vi "Init Module.vi"(7 "Create from class input? (F)":bool, 8 "error in (no error)":errorcluster, 9 "RSI Module in":refnum<class "RSI Module.lvclass">, 10 "Slot Settings":T1, 11 "Module Model":T2) -> (0 "error out":errorcluster, 3 "RSI Module out":refnum<class "RSI Module.lvclass">)   [LabVIEW 2020, in "Modules.lvlib"]
uses:
  Modules.lvlib
  RSI Module/Module Models.ctl
  RSI Module/Slot Settings.ctl
  RSI Module/RSI Module.lvclass
  RSI Module/Channels.ctl
  RSI Module/Channel Type.ctl
  9213/9213.lvclass
  C:/Users/nitest/Desktop/Git 2020/niveristand-scan-engine-module-libraries/Source/RSI Module/RSI Module.lvclass
  9203/9203.lvclass
  9205/9205.lvclass
  9207/9207.lvclass
  9209/9209.lvclass
  9210/9210.lvclass
  9211/9211.lvclass
  9212/9212.lvclass
  9214/9214.lvclass
  9216/9216.lvclass
  9217/9217.lvclass
  9219/9219.lvclass
  9224/9224.lvclass
  9226/9226.lvclass
  9229/9229.lvclass
  9233/9233.lvclass
  9234/9234.lvclass
  9235/9235.lvclass
  9237/9237.lvclass
  9239/9239.lvclass
  9242/9242.lvclass
  9244/9244.lvclass
  9253/9253.lvclass
  9350/9350.lvclass
  9401/9401.lvclass
  9402/9402.lvclass
  9403/9403.lvclass
  9478/9478.lvclass
  SD Module/SD Module.lvclass
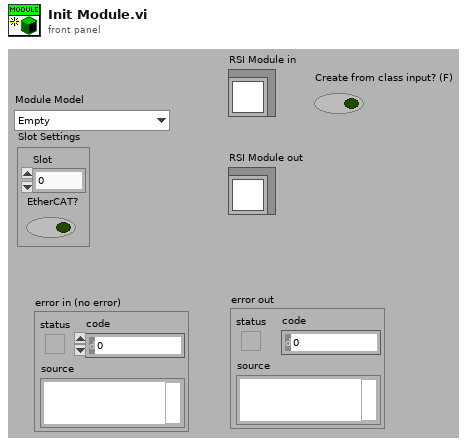
[diagram p1: front panel]
types:
  T1 = typedef "Modules.lvlib/RSI Module.lvclass/Slot Settings.ctl" = cluster{"Slot":u32, "EtherCAT?":bool}
  T2 = typedef "Modules.lvlib/RSI Module.lvclass/Module Models.ctl" = enum16{"Empty", "NI 9201", "NI 9203", "NI 9205", "NI 9206", "NI 9207", "NI 9208", "NI 9209", "NI 9210", "NI 9211", "NI 9212", "NI 9213", "NI 9214", "NI 9215", "NI 9216", "NI 9217", "NI 9219", "NI 9220", "NI 9221", "NI 9222", "NI 9223", "NI 9224", "NI 9225", "NI 9226", "NI 9227", "NI 9228", "NI 9229", "NI 9233", "NI 9234", "NI 9235", "NI 9236", "NI 9237", "NI 9239", "NI 9242", "NI 9244", "NI 9253", "NI 9263", "NI 9264", "NI 9265", "NI 9266", "NI 9269", "NI 9344", "NI 9350", "NI 9375", "NI 9401", "NI 9402", "NI 9403", "NI 9411", "NI 9421", "NI 9422", "NI 9423", "NI 9425", "NI 9426", "NI 9435", "NI 9436", "NI 9437", "NI 9472", "NI 9474", "NI 9475", "NI 9476", "NI 9477", "NI 9478", "NI 9481", "NI 9482", "NI 9485"}
  T3 = typedef "Modules.lvlib/RSI Module.lvclass/Channels.ctl" = cluster{"# Input Channels":i32, "# Output Channels":i32, "Channel Type":T4, "Units":string}
  T4 = typedef "Modules.lvlib/RSI Module.lvclass/Channel Type.ctl" = enum16{"Analog", "Digital"}
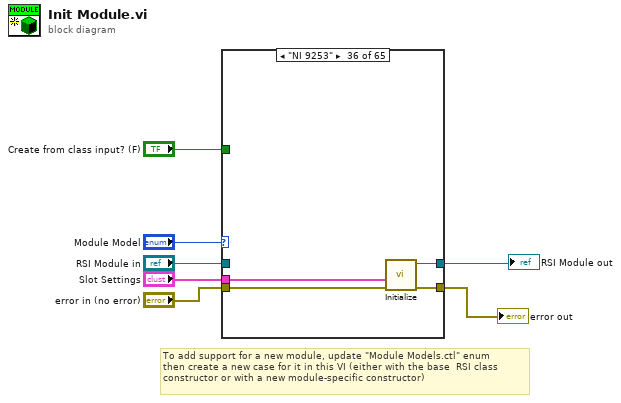
[diagram p0: block diagram]
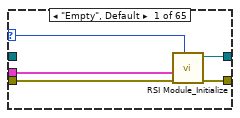
[diagram p2: hidden frame]
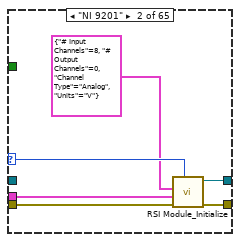
[diagram p3: hidden frame]
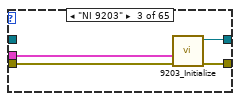
[diagram p4: hidden frame]
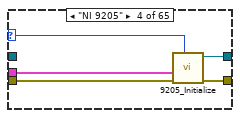
[diagram p5: hidden frame]
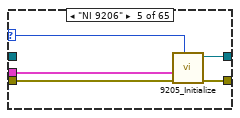
[diagram p6: hidden frame]
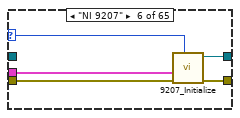
[diagram p7: hidden frame]
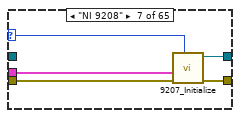
[diagram p8: hidden frame]
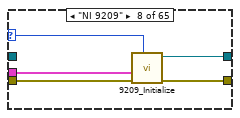
[diagram p9: hidden frame]
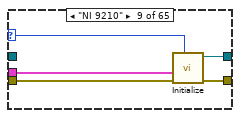
[diagram p10: hidden frame]
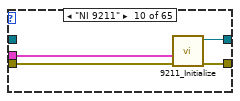
[diagram p11: hidden frame]
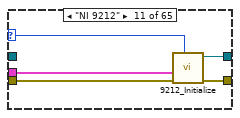
[diagram p12: hidden frame]
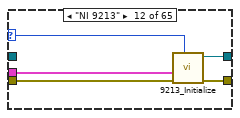
[diagram p13: hidden frame]
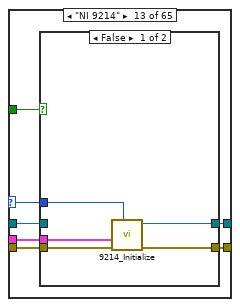
[diagram p14: hidden frame]
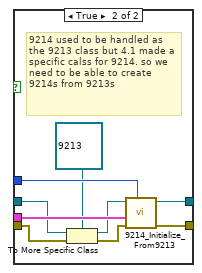
[diagram p15: hidden frame]
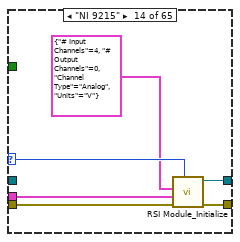
[diagram p16: hidden frame]
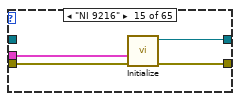
[diagram p17: hidden frame]
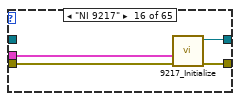
[diagram p18: hidden frame]
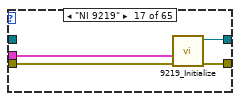
[diagram p19: hidden frame]
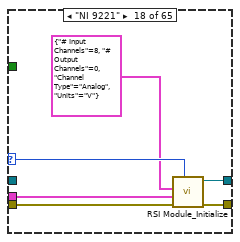
[diagram p20: hidden frame]
diagram:
  # "To add support for a new module, update \"Module Models.ctl\" enum\nthen create a new case for it in this VI (either with the base  RSI class\nconstructor or with a new module-specific constructor)"
  n1 = case shown="\"NI 9253\"" "Module Model" {
    selector: "Module Model" -> [w8 w18 _ w23 w29 w33 w38 w43 w48 _ w57 w62 w69 w93 _ _ _ w111 w117 w123 w129 w134 w140 _ w150 w155 _ _ _ w168 w173 _ _ _ _ _ w203 w209 w215 w221 w227 w233 w235 w244 _ _ _ w263 w279 w297 w317 w338 w344 w347 w366 w386 w404 w421 w442 w464 w470 _ w480 w486 w492]
    tunnel: [w11 w17 w19 w25 w31 w35 w40 w47 w51 w54 w60 w65 w72 w92 w97 w101 w105 w110 w116 w122 w128 w133 w139 w144 w149 w154 w158 w162 w167 w172 w177 w179 w184 w186 w190 w194 w202 w208 w214 w220 w226 w232 w236 w243 w248 w252 w256 w262 w281 w299 w319 w337 w343 w350 w369 w388 w407 w426 w445 w463 w469 w473 w479 w485 w491] -> w3
    tunnel: [w12 w16 w22 w26 w32 w36 w41 w46 w52 w55 w61 w66 w73 w91 w96 w100 w104 w109 w115 w121 w127 w132 w138 w143 w148 w153 w159 w163 w166 w169 w174 w178 w185 w189 w193 w197 w201 w207 w213 w219 w225 w231 w237 w242 w247 w251 w255 w261 w280 w300 w314 w336 w342 w349 w368 w387 w406 w425 w444 w462 w468 w474 w478 w484 w490] -> w6
    tunnel: "Slot Settings" -> [w9 w14 w20 w27 w28 w37 w42 w44 w49 w56 w58 w63 w70 w89 w95 w99 w103 w107 w113 w119 w125 w131 w136 w142 w146 w152 w156 w161 w165 w170 w175 w180 w182 w187 w191 w195 w199 w205 w211 w217 w223 w229 w234 w240 w246 w250 w254 w258 w277 w296 w316 w334 w340 w346 w365 w384 w402 w423 w440 w460 w466 w471 w476 w482 w488]
    tunnel: "error in (no error)" -> [w10 w13 w21 w24 w30 w34 w39 w45 w50 w53 w59 w64 w71 w88 w94 w98 w102 w106 w112 w118 w124 w130 w135 w141 w145 w151 w157 w160 w164 w171 w176 w181 w183 w188 w192 w196 w198 w204 w210 w216 w222 w228 w238 w239 w245 w249 w253 w259 w278 w295 w315 w333 w339 w345 w364 w385 w403 w424 w441 w459 w465 w472 w475 w481 w487]
    tunnel: "Create from class input? (F)" -> [_ _ _ _ _ _ _ _ _ _ _ _ w68 _ _ _ _ _ _ _ _ _ _ _ _ _ _ _ _ _ _ _ _ _ _ _ _ _ _ _ _ _ _ _ _ _ _ _ _ _ _ _ _ _ _ _ _ _ _ _ _ _ _ _ _]
    tunnel: "RSI Module in" -> [_ _ _ _ _ _ _ _ _ _ _ _ w67 _ _ _ _ _ _ _ _ _ _ _ _ _ _ _ _ _ _ _ _ _ _ _ _ _ _ _ _ _ _ _ _ _ _ _ _ _ _ _ _ _ _ _ _ _ _ _ _ _ _ _ _]
    frame "Empty", Default {
      n2 = call "RSI Module_Initialize.vi"("Module Model"=w8, "error in (no error)"=w10, "Slot Settings"=w9) -> ("error out"=w12:errorcluster, "RSI Module out"=w11:refnum<class "RSI Module.lvclass">)  [unwired: 7 in]
    }
    frame "NI 9201" {
      n3 = call "RSI Module_Initialize.vi"("Module Model"=w18, "error in (no error)"=w13, "Slot Settings"=w14, "Channels"=T3 {"# Input Channels"=8, "# Output Channels"=0, "Channel Type"=enum."Analog", "Units"="V"}) -> ("error out"=w16:errorcluster, "RSI Module out"=w17:refnum<class "RSI Module.lvclass">)  [unwired: 6 in]
    }
    frame "NI 9203" {
      n4 = call "9203_Initialize.vi"("error in (no error)"=w21, "Slot Settings"=w20) -> ("error out"=w22:errorcluster, "9203 out"=w19:refnum<class "9203.lvclass">)  [unwired: 8 in]
    }
    frame "NI 9205" {
      n5 = call "9205_Initialize.vi"("Module Model"=w23, "error in (no error)"=w24, "Slot Settings"=w27) -> ("error out"=w26:errorcluster, "9205 out"=w25:refnum<class "9205.lvclass">)  [unwired: 7 in]
    }
    frame "NI 9206" {
      n6 = call "9205_Initialize.vi"("Module Model"=w29, "error in (no error)"=w30, "Slot Settings"=w28) -> ("error out"=w32:errorcluster, "9205 out"=w31:refnum<class "9205.lvclass">)  [unwired: 7 in]
    }
    frame "NI 9207" {
      n7 = call "9207_Initialize.vi"("Module Model"=w33, "error in (no error)"=w34, "Slot Settings"=w37) -> ("error out"=w36:errorcluster, "9207 out"=w35:refnum<class "9207.lvclass">)  [unwired: 7 in]
    }
    frame "NI 9208" {
      n8 = call "9207_Initialize.vi"("Module Model"=w38, "error in (no error)"=w39, "Slot Settings"=w42) -> ("error out"=w41:errorcluster, "9207 out"=w40:refnum<class "9207.lvclass">)  [unwired: 7 in]
    }
    frame "NI 9209" {
      n9 = call "9209_Initialize.vi"("Module Model"=w43, "error in (no error)"=w45, "Slot Settings"=w44) -> ("error out"=w46:errorcluster, "9209 out"=w47:refnum<class "9209.lvclass">)  [unwired: 7 in]
    }
    frame "NI 9210" {
      n10 = call "Initialize.vi"("Module Model"=w48, "error in"=w50, "Slot Settings"=w49) -> ("error out"=w52:errorcluster, "9210 out"=w51:refnum<class "9210.lvclass">)  [unwired: 7 in]
    }
    frame "NI 9211" {
      n11 = call "9211_Initialize.vi"("error in (no error)"=w53, "Slot Settings"=w56) -> ("error out"=w55:errorcluster, "9211 out"=w54:refnum<class "9211.lvclass">)  [unwired: 8 in]
    }
    frame "NI 9212" {
      n12 = call "9212_Initialize.vi"("Module Model"=w57, "error in (no error)"=w59, "Slot Settings"=w58) -> ("error out"=w61:errorcluster, "9213 out"=w60:refnum<class "9212.lvclass">)  [unwired: 7 in]
    }
    frame "NI 9213" {
      n13 = call "9213_Initialize.vi"("Module Model"=w62, "error in (no error)"=w64, "Slot Settings"=w63) -> ("error out"=w66:errorcluster, "9213 out"=w65:refnum<class "9213.lvclass">)  [unwired: 7 in]
    }
    frame "NI 9214" {
      n14 = case shown="False" w68 {
        tunnel: [w78 w87] -> w73
        tunnel: [w77 w86] -> w72
        tunnel: w71 -> [w76 w83]
        tunnel: w70 -> [w75 w85]
        tunnel: w69 -> [w74 w84]
        tunnel: w67 -> [_ w82]
        frame False {
          n15 = call "9214_Initialize.vi"("Module Model"=w74, "error in (no error)"=w76, "Slot Settings"=w75) -> ("error out"=w78:errorcluster, "9214 out"=w77:refnum<class "9214.lvclass">)  [unwired: 7 in]
        }
        frame True {
          # "9214 used to be handled as the 9213 class but 4.1 made a specific calss for 9214. so we need to be able to create 9214s from 9213s"
          n16 = To More Specific Class(target class=refnum<class "9213.lvclass"> refnum ("Modules.lvlib:9213.lvclass"), reference=w82, error in=w83) -> (specific class reference=w80:refnum<class "9213.lvclass">, error out=w79:errorcluster)
          n17 = call "9214_Initialize_From9213.vi"("Module Model"=w84, "error in (no error)"=w79, "Slot Settings"=w85, "9213 in"=w80) -> ("error out"=w87:errorcluster, "9214 out"=w86:refnum<class "9214.lvclass">)  [unwired: 6 in]
        }
      }
    }
    frame "NI 9215" {
      n18 = call "RSI Module_Initialize.vi"("Module Model"=w93, "error in (no error)"=w88, "Slot Settings"=w89, "Channels"=T3 {"# Input Channels"=4, "# Output Channels"=0, "Channel Type"=enum."Analog", "Units"="V"}) -> ("error out"=w91:errorcluster, "RSI Module out"=w92:refnum<class "RSI Module.lvclass">)  [unwired: 6 in]
    }
    frame "NI 9216" {
      n19 = call "Initialize.vi"("error in"=w94, "Slot Settings"=w95) -> ("error out"=w96:errorcluster, "9216 out"=w97:refnum<class "9216.lvclass">)  [unwired: 8 in]
    }
    frame "NI 9217" {
      n20 = call "9217_Initialize.vi"("error in (no error)"=w98, "Slot Settings"=w99) -> ("error out"=w100:errorcluster, "9217 out"=w101:refnum<class "9217.lvclass">)  [unwired: 8 in]
    }
    frame "NI 9219" {
      n21 = call "9219_Initialize.vi"("error in (no error)"=w102, "Slot Settings"=w103) -> ("error out"=w104:errorcluster, "9219 out"=w105:refnum<class "9219.lvclass">)  [unwired: 8 in]
    }
    frame "NI 9221" {
      n22 = call "RSI Module_Initialize.vi"("Module Model"=w111, "error in (no error)"=w106, "Slot Settings"=w107, "Channels"=T3 {"# Input Channels"=8, "# Output Channels"=0, "Channel Type"=enum."Analog", "Units"="V"}) -> ("error out"=w109:errorcluster, "RSI Module out"=w110:refnum<class "RSI Module.lvclass">)  [unwired: 6 in]
    }
    frame "NI 9220" {
      n23 = call "RSI Module_Initialize.vi"("Module Model"=w117, "error in (no error)"=w112, "Slot Settings"=w113, "Channels"=T3 {"# Input Channels"=16, "# Output Channels"=0, "Channel Type"=enum."Analog", "Units"="V"}) -> ("error out"=w115:errorcluster, "RSI Module out"=w116:refnum<class "RSI Module.lvclass">)  [unwired: 6 in]
    }
    frame "NI 9222" {
      n24 = call "RSI Module_Initialize.vi"("Module Model"=w123, "error in (no error)"=w118, "Slot Settings"=w119, "Channels"=T3 {"# Input Channels"=4, "# Output Channels"=0, "Channel Type"=enum."Analog", "Units"="V"}) -> ("error out"=w121:errorcluster, "RSI Module out"=w122:refnum<class "RSI Module.lvclass">)  [unwired: 6 in]
    }
    frame "NI 9223" {
      n25 = call "RSI Module_Initialize.vi"("Module Model"=w129, "error in (no error)"=w124, "Slot Settings"=w125, "Channels"=T3 {"# Input Channels"=4, "# Output Channels"=0, "Channel Type"=enum."Analog", "Units"="V"}) -> ("error out"=w127:errorcluster, "RSI Module out"=w128:refnum<class "RSI Module.lvclass">)  [unwired: 6 in]
    }
    frame "NI 9224" {
      n26 = call "9224_Initialize.vi"("Module Model"=w134, "error in (no error)"=w130, "Slot Settings"=w131) -> ("error out"=w132:errorcluster, "9224 out"=w133:refnum<class "9224.lvclass">)  [unwired: 7 in]
    }
    frame "NI 9225" {
      n27 = call "RSI Module_Initialize.vi"("Module Model"=w140, "error in (no error)"=w135, "Slot Settings"=w136, "Channels"=T3 {"# Input Channels"=3, "# Output Channels"=0, "Channel Type"=enum."Analog", "Units"="Vrms"}) -> ("error out"=w138:errorcluster, "RSI Module out"=w139:refnum<class "RSI Module.lvclass">)  [unwired: 6 in]
    }
    frame "NI 9226" {
      n28 = call "Initialize.vi"("error in"=w141, "Slot Settings"=w142) -> ("error out"=w143:errorcluster, "9226 out"=w144:refnum<class "9226.lvclass">)  [unwired: 8 in]
    }
    frame "NI 9227" {
      n29 = call "RSI Module_Initialize.vi"("Module Model"=w150, "error in (no error)"=w145, "Slot Settings"=w146, "Channels"=T3 {"# Input Channels"=4, "# Output Channels"=0, "Channel Type"=enum."Analog", "Units"="Arms"}) -> ("error out"=w148:errorcluster, "RSI Module out"=w149:refnum<class "RSI Module.lvclass">)  [unwired: 6 in]
    }
    frame "NI 9228" {
      n30 = call "9224_Initialize.vi"("Module Model"=w155, "error in (no error)"=w151, "Slot Settings"=w152) -> ("error out"=w153:errorcluster, "9224 out"=w154:refnum<class "9224.lvclass">)  [unwired: 7 in]
    }
    frame "NI 9229" {
      n31 = call "9229_Initialize.vi"("error in (no error)"=w157, "Slot Settings"=w156) -> ("error out"=w159:errorcluster, "9229 out"=w158:refnum<class "9229.lvclass">)  [unwired: 8 in]
    }
    frame "NI 9233" {
      n32 = call "9233_Initialize.vi"("error in (no error)"=w160, "Slot Settings"=w161) -> ("error out"=w163:errorcluster, "9233 out"=w162:refnum<class "9233.lvclass">)  [unwired: 8 in]
    }
    frame "NI 9234" {
      n33 = call "9234_Initialize.vi"("error in (no error)"=w164, "Slot Settings"=w165) -> ("error out"=w166:errorcluster, "9234 out"=w167:refnum<class "9234.lvclass">)  [unwired: 8 in]
    }
    frame "NI 9235" {
      n34 = call "9235_Initialize.vi"("Module Model"=w168, "error in (no error)"=w171, "Slot Settings"=w170) -> ("error out"=w169:errorcluster, "9235 out"=w172:refnum<class "9235.lvclass">)  [unwired: 7 in]
    }
    frame "NI 9236" {
      n35 = call "9235_Initialize.vi"("Module Model"=w173, "error in (no error)"=w176, "Slot Settings"=w175) -> ("error out"=w174:errorcluster, "9235 out"=w177:refnum<class "9235.lvclass">)  [unwired: 7 in]
    }
    frame "NI 9237" {
      n36 = call "9237_Initialize.vi"("error in (no error)"=w181, "Slot Settings"=w180) -> ("error out"=w178:errorcluster, "9237 out"=w179:refnum<class "9237.lvclass">)  [unwired: 8 in]
    }
    frame "NI 9239" {
      n37 = call "9239_Initialize.vi"("error in (no error)"=w183, "Slot Settings"=w182) -> ("error out"=w185:errorcluster, "9239 out"=w184:refnum<class "9239.lvclass">)  [unwired: 8 in]
    }
    frame "NI 9242" {
      n38 = call "9242_Initialize.vi"("error in (no error)"=w188, "Slot Settings"=w187) -> ("error out"=w189:errorcluster, "Modules.lvlib:9242.lvclass"=w186:refnum<class "9242.lvclass">)  [unwired: 8 in]
    }
    frame "NI 9244" {
      n39 = call "9244_Initialize.vi"("error in (no error)"=w192, "Slot Settings"=w191) -> ("error out"=w193:errorcluster, "Modules.lvlib:9244.lvclass"=w190:refnum<class "9244.lvclass">)  [unwired: 8 in]
    }
    frame "NI 9253" {
      n40 = call "Initialize.vi"("error in"=w196, "Slot Settings"=w195) -> ("error out"=w197:errorcluster, "9253 out"=w194:refnum<class "9253.lvclass">)  [unwired: 8 in]
    }
    frame "NI 9263" {
      n41 = call "RSI Module_Initialize.vi"("Module Model"=w203, "error in (no error)"=w198, "Slot Settings"=w199, "Channels"=T3 {"# Input Channels"=0, "# Output Channels"=4, "Channel Type"=enum."Analog", "Units"="V"}) -> ("error out"=w201:errorcluster, "RSI Module out"=w202:refnum<class "RSI Module.lvclass">)  [unwired: 6 in]
    }
    frame "NI 9264" {
      n42 = call "RSI Module_Initialize.vi"("Module Model"=w209, "error in (no error)"=w204, "Slot Settings"=w205, "Channels"=T3 {"# Input Channels"=0, "# Output Channels"=16, "Channel Type"=enum."Analog", "Units"="V"}) -> ("error out"=w207:errorcluster, "RSI Module out"=w208:refnum<class "RSI Module.lvclass">)  [unwired: 6 in]
    }
    frame "NI 9265" {
      n43 = call "RSI Module_Initialize.vi"("Module Model"=w215, "error in (no error)"=w210, "Slot Settings"=w211, "Channels"=T3 {"# Input Channels"=0, "# Output Channels"=4, "Channel Type"=enum."Analog", "Units"="A"}) -> ("error out"=w213:errorcluster, "RSI Module out"=w214:refnum<class "RSI Module.lvclass">)  [unwired: 6 in]
    }
    frame "NI 9266" {
      n44 = call "RSI Module_Initialize.vi"("Module Model"=w221, "error in (no error)"=w216, "Slot Settings"=w217, "Channels"=T3 {"# Input Channels"=0, "# Output Channels"=8, "Channel Type"=enum."Analog", "Units"="A"}) -> ("error out"=w219:errorcluster, "RSI Module out"=w220:refnum<class "RSI Module.lvclass">)  [unwired: 6 in]
    }
    frame "NI 9269" {
      n45 = call "RSI Module_Initialize.vi"("Module Model"=w227, "error in (no error)"=w222, "Slot Settings"=w223, "Channels"=T3 {"# Input Channels"=0, "# Output Channels"=4, "Channel Type"=enum."Analog", "Units"="V"}) -> ("error out"=w225:errorcluster, "RSI Module out"=w226:refnum<class "RSI Module.lvclass">)  [unwired: 6 in]
    }
    frame "NI 9344" {
      n46 = call "RSI Module_Initialize.vi"("Module Model"=w233, "error in (no error)"=w228, "Slot Settings"=w229, "Channels"=T3 {"# Input Channels"=4, "# Output Channels"=4, "Channel Type"=enum."Digital", "Units"=""}) -> ("error out"=w231:errorcluster, "RSI Module out"=w232:refnum<class "RSI Module.lvclass">)  [unwired: 6 in]
    }
    frame "NI 9350" {
      n47 = call "9350_Initialize.vi"("Module Model"=w235, "error in (no error)"=w238, "Slot Settings"=w234) -> ("error out"=w237:errorcluster, "9350 out"=w236:refnum<class "9350.lvclass">)  [unwired: 7 in]
    }
    frame "NI 9375" {
      n48 = call "RSI Module_Initialize.vi"("Module Model"=w244, "error in (no error)"=w239, "Slot Settings"=w240, "Channels"=T3 {"# Input Channels"=16, "# Output Channels"=16, "Channel Type"=enum."Digital", "Units"=""}) -> ("error out"=w242:errorcluster, "RSI Module out"=w243:refnum<class "RSI Module.lvclass">)  [unwired: 6 in]
    }
    frame "NI 9401" {
      n49 = call "9401_Initialize.vi"("error in (no error)"=w245, "Slot Settings"=w246) -> ("error out"=w247:errorcluster, "9401 out"=w248:refnum<class "9401.lvclass">)  [unwired: 8 in]
    }
    frame "NI 9402" {
      n50 = call "9402_Initialize.vi"("error in (no error)"=w249, "Slot Settings"=w250) -> ("error out"=w251:errorcluster, "9402 out"=w252:refnum<class "9402.lvclass">)  [unwired: 8 in]
    }
    frame "NI 9403" {
      n51 = call "9403_Initialize.vi"("error in (no error)"=w253, "Slot Settings"=w254) -> ("error out"=w255:errorcluster, "9403 out"=w256:refnum<class "9403.lvclass">)  [unwired: 8 in]
    }
    frame "NI 9411" {
      n52 = Unbundle By Name(w258) -> ("EtherCAT?"=w257:bool)
      n53 = case shown="True" w257 {
        tunnel: w263 -> [w269 w272]
        tunnel: [w268 w273] -> w262
        tunnel: [w267 w274] -> w261
        tunnel: T3 {"# Input Channels"=6, "# Output Channels"=0, "Channel Type"=enum."Digital", "Units"=""} ("Channels") -> [w266 w271]
        tunnel: w259 -> [w265 w275]
        tunnel: w258 -> [w264 w270]
        frame False {
          n54 = call "SD Module_Initialize.vi"("Module Model"=w269, "error in (no error)"=w265, "Slot Settings"=w264, "Channels"=w266) -> ("error out"=w267:errorcluster, "SD Module out"=w268:refnum<class "SD Module.lvclass">)  [unwired: 6 in]
        }
        frame True {
          n55 = call "RSI Module_Initialize.vi"("Module Model"=w272, "error in (no error)"=w275, "Slot Settings"=w270, "Channels"=w271) -> ("error out"=w274:errorcluster, "RSI Module out"=w273:refnum<class "RSI Module.lvclass">)  [unwired: 6 in]
        }
      }
    }
    frame "NI 9421" {
      n56 = Unbundle By Name(w277) -> ("EtherCAT?"=w282:bool)
      n57 = case shown="True" w282 {
        tunnel: w279 -> [w288 w291]
        tunnel: [w287 w292] -> w281
        tunnel: [w286 w293] -> w280
        tunnel: T3 {"# Input Channels"=8, "# Output Channels"=0, "Channel Type"=enum."Digital", "Units"=""} ("Channels") -> [w285 w290]
        tunnel: w278 -> [w284 w294]
        tunnel: w277 -> [w283 w289]
        frame False {
          n58 = call "SD Module_Initialize.vi"("Module Model"=w288, "error in (no error)"=w284, "Slot Settings"=w283, "Channels"=w285) -> ("error out"=w286:errorcluster, "SD Module out"=w287:refnum<class "SD Module.lvclass">)  [unwired: 6 in]
        }
        frame True {
          n59 = call "RSI Module_Initialize.vi"("Module Model"=w291, "error in (no error)"=w294, "Slot Settings"=w289, "Channels"=w290) -> ("error out"=w293:errorcluster, "RSI Module out"=w292:refnum<class "RSI Module.lvclass">)  [unwired: 6 in]
        }
      }
    }
    frame "NI 9422" {
      n60 = Unbundle By Name(w296) -> ("EtherCAT?"=w301:bool)
      n61 = case shown="True" w301 {
        tunnel: w297 -> [w307 w310]
        tunnel: [w306 w311] -> w299
        tunnel: [w305 w312] -> w300
        tunnel: T3 {"# Input Channels"=8, "# Output Channels"=0, "Channel Type"=enum."Digital", "Units"=""} ("Channels") -> [w304 w309]
        tunnel: w295 -> [w303 w313]
        tunnel: w296 -> [w302 w308]
        frame False {
          n62 = call "SD Module_Initialize.vi"("Module Model"=w307, "error in (no error)"=w303, "Slot Settings"=w302, "Channels"=w304) -> ("error out"=w305:errorcluster, "SD Module out"=w306:refnum<class "SD Module.lvclass">)  [unwired: 6 in]
        }
        frame True {
          n63 = call "RSI Module_Initialize.vi"("Module Model"=w310, "error in (no error)"=w313, "Slot Settings"=w308, "Channels"=w309) -> ("error out"=w312:errorcluster, "RSI Module out"=w311:refnum<class "RSI Module.lvclass">)  [unwired: 6 in]
        }
      }
    }
    frame "NI 9423" {
      n64 = Unbundle By Name(w316) -> ("EtherCAT?"=w320:bool)
      n65 = case shown="False" w320 {
        tunnel: w317 -> [w326 w329]
        tunnel: [w325 w330] -> w319
        tunnel: [w324 w331] -> w314
        tunnel: T3 {"# Input Channels"=8, "# Output Channels"=0, "Channel Type"=enum."Digital", "Units"=""} ("Channels") -> [w323 w328]
        tunnel: w315 -> [w322 w332]
        tunnel: w316 -> [w321 w327]
        frame False {
          n66 = call "SD Module_Initialize.vi"("Module Model"=w326, "error in (no error)"=w322, "Slot Settings"=w321, "Channels"=w323) -> ("error out"=w324:errorcluster, "SD Module out"=w325:refnum<class "SD Module.lvclass">)  [unwired: 6 in]
        }
        frame True {
          n67 = call "RSI Module_Initialize.vi"("Module Model"=w329, "error in (no error)"=w332, "Slot Settings"=w327, "Channels"=w328) -> ("error out"=w331:errorcluster, "RSI Module out"=w330:refnum<class "RSI Module.lvclass">)  [unwired: 6 in]
        }
      }
    }
    frame "NI 9425" {
      n68 = call "RSI Module_Initialize.vi"("Module Model"=w338, "error in (no error)"=w333, "Slot Settings"=w334, "Channels"=T3 {"# Input Channels"=32, "# Output Channels"=0, "Channel Type"=enum."Digital", "Units"=""}) -> ("error out"=w336:errorcluster, "RSI Module out"=w337:refnum<class "RSI Module.lvclass">)  [unwired: 6 in]
    }
    frame "NI 9426" {
      n69 = call "RSI Module_Initialize.vi"("Module Model"=w344, "error in (no error)"=w339, "Slot Settings"=w340, "Channels"=T3 {"# Input Channels"=32, "# Output Channels"=0, "Channel Type"=enum."Digital", "Units"=""}) -> ("error out"=w342:errorcluster, "RSI Module out"=w343:refnum<class "RSI Module.lvclass">)  [unwired: 6 in]
    }
    frame "NI 9435" {
      n70 = Unbundle By Name(w346) -> ("EtherCAT?"=w351:bool)
      n71 = case shown="True" w351 {
        tunnel: w347 -> [w357 w360]
        tunnel: [w356 w361] -> w350
        tunnel: [w355 w362] -> w349
        tunnel: T3 {"# Input Channels"=4, "# Output Channels"=0, "Channel Type"=enum."Digital", "Units"=""} ("Channels") -> [w354 w359]
        tunnel: w345 -> [w353 w363]
        tunnel: w346 -> [w352 w358]
        frame False {
          n72 = call "SD Module_Initialize.vi"("Module Model"=w357, "error in (no error)"=w353, "Slot Settings"=w352, "Channels"=w354) -> ("error out"=w355:errorcluster, "SD Module out"=w356:refnum<class "SD Module.lvclass">)  [unwired: 6 in]
        }
        frame True {
          n73 = call "RSI Module_Initialize.vi"("Module Model"=w360, "error in (no error)"=w363, "Slot Settings"=w358, "Channels"=w359) -> ("error out"=w362:errorcluster, "RSI Module out"=w361:refnum<class "RSI Module.lvclass">)  [unwired: 6 in]
        }
      }
    }
    frame "NI 9436" {
      n74 = Unbundle By Name(w365) -> ("EtherCAT?"=w370:bool)
      n75 = case shown="False" w370 {
        tunnel: w366 -> [w376 w379]
        tunnel: [w375 w380] -> w369
        tunnel: [w374 w381] -> w368
        tunnel: T3 {"# Input Channels"=8, "# Output Channels"=0, "Channel Type"=enum."Digital", "Units"=""} ("Channels") -> [w373 w378]
        tunnel: w364 -> [w372 w382]
        tunnel: w365 -> [w371 w377]
        frame False {
          n76 = call "SD Module_Initialize.vi"("Module Model"=w376, "error in (no error)"=w372, "Slot Settings"=w371, "Channels"=w373) -> ("error out"=w374:errorcluster, "SD Module out"=w375:refnum<class "SD Module.lvclass">)  [unwired: 6 in]
        }
        frame True {
          n77 = call "RSI Module_Initialize.vi"("Module Model"=w379, "error in (no error)"=w382, "Slot Settings"=w377, "Channels"=w378) -> ("error out"=w381:errorcluster, "RSI Module out"=w380:refnum<class "RSI Module.lvclass">)  [unwired: 6 in]
        }
      }
    }
    frame "NI 9437" {
      n78 = Unbundle By Name(w384) -> ("EtherCAT?"=w389:bool)
      n79 = case shown="True" w389 {
        tunnel: w386 -> [w395 w398]
        tunnel: [w394 w399] -> w388
        tunnel: [w393 w400] -> w387
        tunnel: T3 {"# Input Channels"=8, "# Output Channels"=0, "Channel Type"=enum."Digital", "Units"=""} ("Channels") -> [w392 w397]
        tunnel: w385 -> [w391 w401]
        tunnel: w384 -> [w390 w396]
        frame False {
          n80 = call "SD Module_Initialize.vi"("Module Model"=w395, "error in (no error)"=w391, "Slot Settings"=w390, "Channels"=w392) -> ("error out"=w393:errorcluster, "SD Module out"=w394:refnum<class "SD Module.lvclass">)  [unwired: 6 in]
        }
        frame True {
          n81 = call "RSI Module_Initialize.vi"("Module Model"=w398, "error in (no error)"=w401, "Slot Settings"=w396, "Channels"=w397) -> ("error out"=w400:errorcluster, "RSI Module out"=w399:refnum<class "RSI Module.lvclass">)  [unwired: 6 in]
        }
      }
    }
    frame "NI 9472" {
      n82 = Unbundle By Name(w402) -> ("EtherCAT?"=w408:bool)
      n83 = case shown="True" w408 {
        tunnel: w404 -> [w414 w417]
        tunnel: [w413 w418] -> w407
        tunnel: [w412 w419] -> w406
        tunnel: T3 {"# Input Channels"=0, "# Output Channels"=8, "Channel Type"=enum."Digital", "Units"=""} ("Channels") -> [w411 w416]
        tunnel: w403 -> [w410 w420]
        tunnel: w402 -> [w409 w415]
        frame False {
          n84 = call "SD Module_Initialize.vi"("Module Model"=w414, "error in (no error)"=w410, "Slot Settings"=w409, "Channels"=w411) -> ("error out"=w412:errorcluster, "SD Module out"=w413:refnum<class "SD Module.lvclass">)  [unwired: 6 in]
        }
        frame True {
          n85 = call "RSI Module_Initialize.vi"("Module Model"=w417, "error in (no error)"=w420, "Slot Settings"=w415, "Channels"=w416) -> ("error out"=w419:errorcluster, "RSI Module out"=w418:refnum<class "RSI Module.lvclass">)  [unwired: 6 in]
        }
      }
    }
    frame "NI 9474" {
      n86 = Unbundle By Name(w423) -> ("EtherCAT?"=w427:bool)
      n87 = case shown="False" w427 {
        tunnel: w421 -> [w433 w436]
        tunnel: [w432 w437] -> w426
        tunnel: [w431 w438] -> w425
        tunnel: T3 {"# Input Channels"=0, "# Output Channels"=8, "Channel Type"=enum."Digital", "Units"=""} ("Channels") -> [w430 w435]
        tunnel: w424 -> [w429 w439]
        tunnel: w423 -> [w428 w434]
        frame False {
          n88 = call "SD Module_Initialize.vi"("Module Model"=w433, "error in (no error)"=w429, "Slot Settings"=w428, "Channels"=w430) -> ("error out"=w431:errorcluster, "SD Module out"=w432:refnum<class "SD Module.lvclass">)  [unwired: 6 in]
        }
        frame True {
          n89 = call "RSI Module_Initialize.vi"("Module Model"=w436, "error in (no error)"=w439, "Slot Settings"=w434, "Channels"=w435) -> ("error out"=w438:errorcluster, "RSI Module out"=w437:refnum<class "RSI Module.lvclass">)  [unwired: 6 in]
        }
      }
    }
    frame "NI 9475" {
      n90 = Unbundle By Name(w440) -> ("EtherCAT?"=w446:bool)
      n91 = case shown="True" w446 {
        tunnel: w442 -> [w452 w455]
        tunnel: [w451 w456] -> w445
        tunnel: [w450 w457] -> w444
        tunnel: T3 {"# Input Channels"=0, "# Output Channels"=8, "Channel Type"=enum."Digital", "Units"=""} ("Channels") -> [w449 w454]
        tunnel: w441 -> [w448 w458]
        tunnel: w440 -> [w447 w453]
        frame False {
          n92 = call "SD Module_Initialize.vi"("Module Model"=w452, "error in (no error)"=w448, "Slot Settings"=w447, "Channels"=w449) -> ("error out"=w450:errorcluster, "SD Module out"=w451:refnum<class "SD Module.lvclass">)  [unwired: 6 in]
        }
        frame True {
          n93 = call "RSI Module_Initialize.vi"("Module Model"=w455, "error in (no error)"=w458, "Slot Settings"=w453, "Channels"=w454) -> ("error out"=w457:errorcluster, "RSI Module out"=w456:refnum<class "RSI Module.lvclass">)  [unwired: 6 in]
        }
      }
    }
    frame "NI 9476" {
      n94 = call "RSI Module_Initialize.vi"("Module Model"=w464, "error in (no error)"=w459, "Slot Settings"=w460, "Channels"=T3 {"# Input Channels"=0, "# Output Channels"=32, "Channel Type"=enum."Digital", "Units"=""}) -> ("error out"=w462:errorcluster, "RSI Module out"=w463:refnum<class "RSI Module.lvclass">)  [unwired: 6 in]
    }
    frame "NI 9477" {
      n95 = call "RSI Module_Initialize.vi"("Module Model"=w470, "error in (no error)"=w465, "Slot Settings"=w466, "Channels"=T3 {"# Input Channels"=0, "# Output Channels"=32, "Channel Type"=enum."Digital", "Units"=""}) -> ("error out"=w468:errorcluster, "RSI Module out"=w469:refnum<class "RSI Module.lvclass">)  [unwired: 6 in]
    }
    frame "NI 9478" {
      n96 = call "9478_Initialize.vi"("error in (no error)"=w472, "Slot Settings"=w471) -> ("error out"=w474:errorcluster, "9478 out"=w473:refnum<class "9478.lvclass">)  [unwired: 8 in]
    }
    frame "NI 9481" {
      n97 = call "RSI Module_Initialize.vi"("Module Model"=w480, "error in (no error)"=w475, "Slot Settings"=w476, "Channels"=T3 {"# Input Channels"=0, "# Output Channels"=4, "Channel Type"=enum."Digital", "Units"=""}) -> ("error out"=w478:errorcluster, "RSI Module out"=w479:refnum<class "RSI Module.lvclass">)  [unwired: 6 in]
    }
    frame "NI 9482" {
      n98 = call "RSI Module_Initialize.vi"("Module Model"=w486, "error in (no error)"=w481, "Slot Settings"=w482, "Channels"=T3 {"# Input Channels"=0, "# Output Channels"=4, "Channel Type"=enum."Digital", "Units"=""}) -> ("error out"=w484:errorcluster, "RSI Module out"=w485:refnum<class "RSI Module.lvclass">)  [unwired: 6 in]
    }
    frame "NI 9485" {
      n99 = call "RSI Module_Initialize.vi"("Module Model"=w492, "error in (no error)"=w487, "Slot Settings"=w488, "Channels"=T3 {"# Input Channels"=0, "# Output Channels"=8, "Channel Type"=enum."Digital", "Units"=""}) -> ("error out"=w490:errorcluster, "RSI Module out"=w491:refnum<class "RSI Module.lvclass">)  [unwired: 6 in]
    }
  }
  "error out" <- w6
  "RSI Module out" <- w3
